vi "RemoteVI Process Path.vi"(0 "process ID":u32) -> (4 "path":string)   [LabVIEW 2020, in "RemoteVI.lvlib"]
doc: "The full path of the program process ID runs (kernel32 OpenProcess.vi with PROCESS_QUERY_LIMITED_INFORMATION, kernel32 QueryFullProcessImageNameW.vi, kernel32 CloseHandle.vi), UTF-16 narrowed to bytes (Latin-1; other characters become ?). Empty when the process cannot be opened (another user's or a protected process). Errors of the calls are not reported."
uses:
  RemoteVI.lvlib
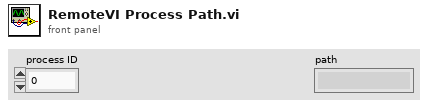
[diagram p1: front panel]
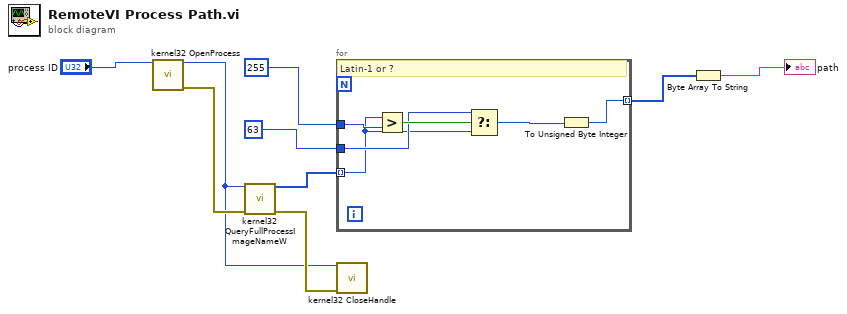
[diagram p0: block diagram]
diagram:
  n1 = call "kernel32 OpenProcess.vi"("process ID"="process ID") -> ("HANDLE"=w2:u64, "error out"=w3:errorcluster)  [unwired: 13 in]
  n2 = call "kernel32 QueryFullProcessImageNameW.vi"("hProcess"=w2, "error in"=w3) -> ("path"=w4:u16[], "error out"=w5:errorcluster)  [unwired: 11 in, 1 out]
  n3 = for {
    tunnel: u16 255 -> [w11]
    tunnel: u16 63 -> [w12]
    tunnel: w4 -> [w10] mode=indexing
    tunnel: [w15] -> w8 mode=indexing
    # "Latin-1 or ?"
    n4 = Greater?(x=w10, y=w11) -> (0:w13:bool)
    n5 = Select(t=w12, s=w13, f=w10) -> (s? t:f=w14:u16)
    n6 = To Unsigned Byte Integer(number=w14) -> (unsigned 8bit integer=w15:u8)
  }
  n7 = call "kernel32 CloseHandle.vi"("hObject"=w2, "error in"=w5) -> ()  [unwired: 12 in, 2 out]
  n8 = Byte Array To String(unsigned byte array=w8) -> (string=→"path":string)
